vi "GOOP_TcpIpListener.vi"() -> ()   [LabVIEW 2020]
uses:
  <resource>/Framework/Providers/Open_GDS/SubVIs/GOOP_UMLEditor_CallMainAction.ctl
panel:
  out "Response":cluster{"action":string, "file":string}
  out "Header":string
  out "error out":errorcluster
  out "Body":string
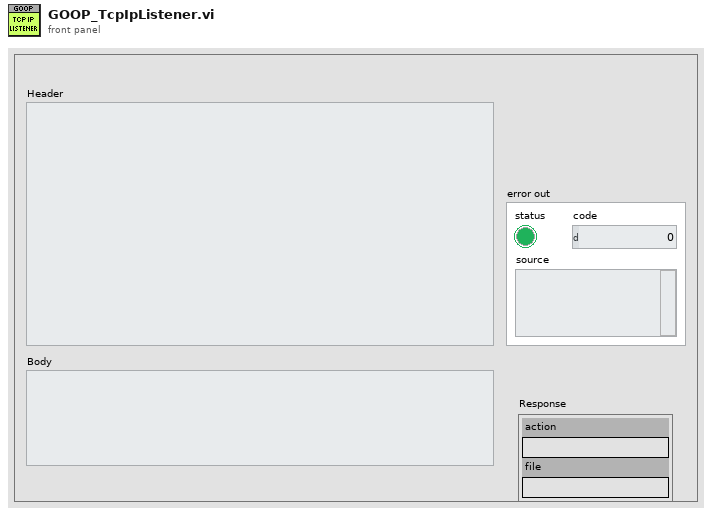
[diagram p1: front panel]
types:
  T1 = enum16{"Standard", "Buffered", "CRLF", "Immediate"}
  T2 = typedef "GOOP_UMLEditor_CallMainAction.ctl" = enum16{"OpenUmlEditor", "ReverseEngineering:WholeProject", "ReverseEngineering:OneClass", "ReverseEngineering:OneVI", "ShowInStateDiagram:OneVI", "OpenUMLFile"}
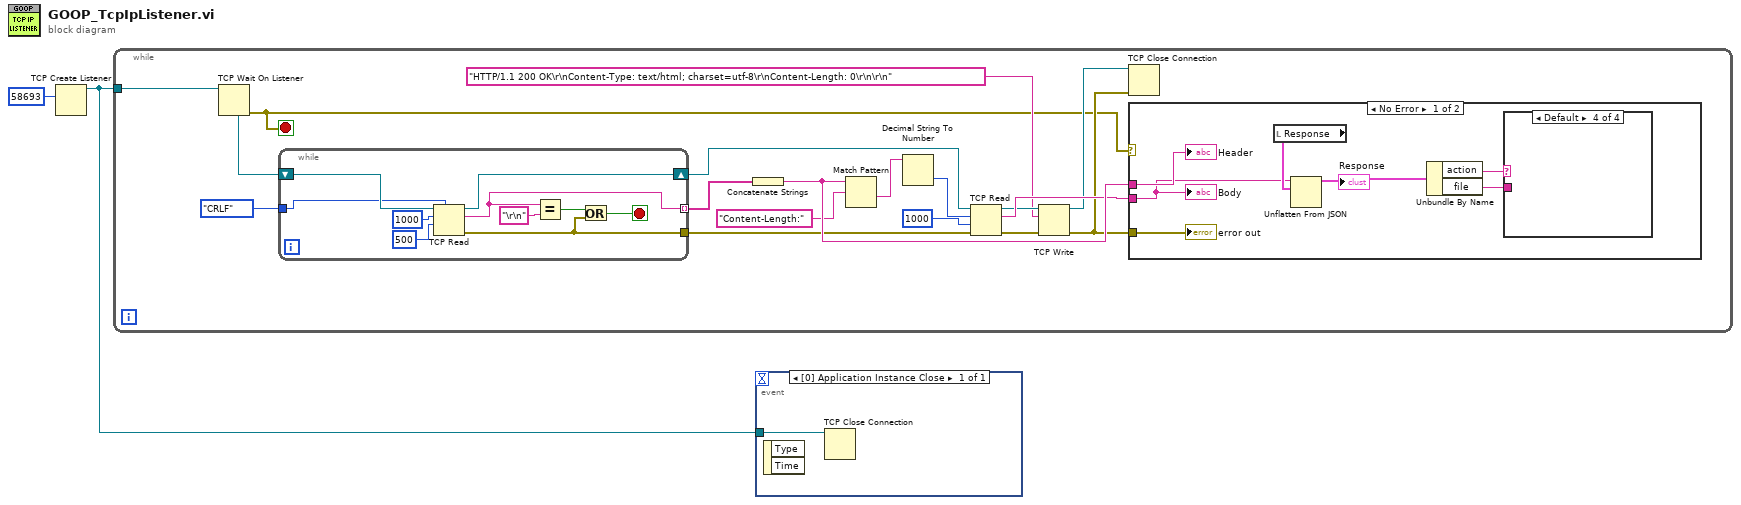
[diagram p0: block diagram]
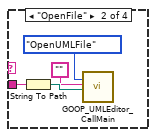
[diagram p3: hidden frame]
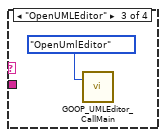
[diagram p4: hidden frame]
diagram:
  n1 = TCP Create Listener(10:u16 58693 ("port")) -> (3:w2:refnum<k5>)  [unwired: 4 in, 2 out]
  n2 = while {
    tunnel: w2 -> [w20]
    stop <- w3 stop-if-true
    n3 = TCP Wait On Listener(11:w20) -> (0:w3:errorcluster, 4:w19:refnum<k5>)  [unwired: 3 in, 3 out]
    n4 = while {
      tunnel: T1."CRLF" ("mode (standard)") -> [w41]
      tunnel: [w37] -> w17 mode=indexing
      tunnel: [w35] -> w13
      shift-right: [w38] -> w7
      shift-left: w19 -> [w42]
      stop <- w34 stop-if-true
      n5 = TCP Read(connection ID=w42, bytes to read=1000, 7:w41, 9:500 ("timeout ms (25000)")) -> (connection ID out=w38:refnum<k5>, data out=w37:string, error out=w35:errorcluster)  [unwired: 1 in]
      n6 = Equal?(x=w37, y="\r\n") -> (x = y?=w33:bool)
      n7 = Or(x=w33, y=w35) -> (x .or. y?=w34:bool)
    }
    n8 = Concatenate Strings(w17) -> (w16:string)
    n9 = Match Pattern(string=w16, regular expression="Content-Length:") -> (after substring=w14:string)  [unwired: 1 in, 3 out]
    n10 = Decimal String To Number(string=w14) -> (number=w12:i32)  [unwired: 2 in, 1 out]
    n11 = TCP Read(connection ID=w7, bytes to read=w12, error in (no error)=w13, 9:1000 ("timeout ms (25000)")) -> (connection ID out=w9:refnum<k5>, data out=w10:string, error out=w4:errorcluster)  [unwired: 1 in]
    n12 = TCP Write(connection ID=w9, data in="HTTP/1.1 200 OK\r\nContent-Type: text/html; charset=utf-8\r\nContent-Length: 0\r\n\r\n", error in (no error)=w4) -> (connection ID out=w6:refnum<k5>, error out=w8:errorcluster)  [unwired: 1 in, 1 out]
    n13 = TCP Close Connection(connection ID=w6, error in (no error)=w8) -> ()  [unwired: 1 in, 2 out]
    n14 = case shown="No Error" w3 {
      tunnel: w8 -> [w27 _]
      tunnel: w16 -> [w26 _]
      tunnel: w10 -> [w24 _]
      frame No Error {
        n15 = local read "Response"() -> (w25:cluster{"action":string, "file":string})
        n16 = Unflatten From JSON(JSON string=w24, type and defaults=w25) -> (value=w23:cluster{"action":string, "file":string})  [unwired: 5 in, 1 out]
        "Response" <- w23
        n17 = Unbundle By Name(w23) -> ("action"=w22:string, "file"=w21:string)
        n18 = case shown="Default" w22 {
          tunnel: w21 -> [_ w31 _ _]
          frame "False" {
          }
          frame "OpenFile" {
            n19 = String To Path(string=w31) -> (path=w30:path)
            n20 = call <resource>:"GOOP_UMLEditor_CallMain.vi"("Enum"=GOOP_UMLEditor_CallMainAction."OpenUMLFile", "Project"="", "Class/VI-Path"=w30) -> ()  [unwired: 16 in, 1 out]
          }
          frame "OpenUMLEditor" {
            n21 = call <resource>:"GOOP_UMLEditor_CallMain.vi"("Enum"=GOOP_UMLEditor_CallMainAction."OpenUmlEditor") -> ()  [unwired: 18 in, 1 out]
          }
          frame Default {
          }
        }
        "Header" <- w26
        "error out" <- w27
        "Body" <- w24
      }
      frame Error {
      }
    }
  }
  n22 = event shown="[0] Application Instance Close" {
    selector: _ -> [_]
    dyn-events: _ -> [_]
    timeout: _ -> [_]
    tunnel: w2 -> [w43]
    event Application Instance Close {
      n23 = event-data() -> ()  [unwired: 1 in, 2 out]
      n24 = TCP Close Connection(connection ID=w43) -> ()  [unwired: 2 in, 2 out]
    }
  }
